vi "get supported types.vi"(8 "error in":errorcluster, 11 "module configuration in":refnum<class "base TBM sequencer configuration.lvclass">) -> (0 "error out":errorcluster, 2 "supported types":T1[](array[typedef]), 3 "module configuration out":refnum<class "base TBM sequencer configuration.lvclass">)   [LabVIEW 2015, in "base TBM sequencer configuration.lvclass"]
doc: "Provides an interface for determining the targets supported by a given configuration/runtime class pairing. This should be overridden by any useful child class."
uses:
  base TBM sequencer configuration.lvclass
  <vilib>/NI/Tag Bus/tag/Data Type.ctl
  <vilib>/NI/Tag Bus Module Framework/module configuration/TBM module configuration.lvclass
  <vilib>/NI/Tag Bus/tag/tag descriptor.lvclass
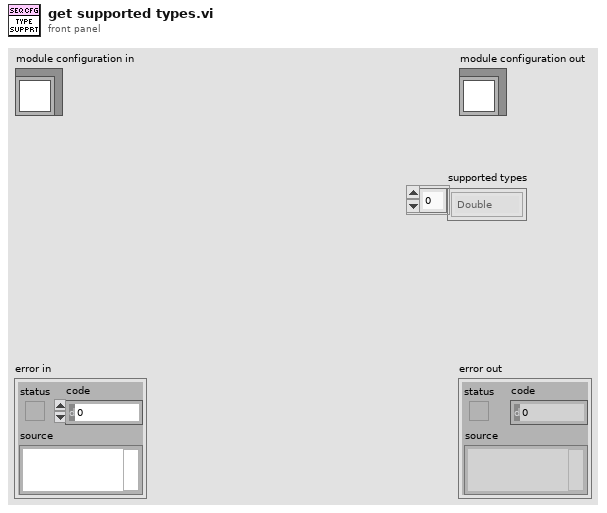
[diagram p1: front panel]
types:
  T1 = typedef "tag bus.lvlib/tag descriptor.lvclass/Data Type.ctl" = enum16{"Double", "Single", "I64", "I32", "I16", "I8", "U64", "U32", "U16", "U8", "Boolean", "String", "Array of Double", "Array of Single", "Array of I64", "Array of I32", "Array of I16", "Array of I8", "Array of U64", "Array of U32", "Array of U16", "Array of U8", "Array of Boolean", "Array of String"}
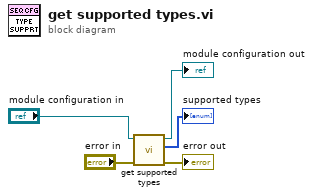
[diagram p0: block diagram]
diagram:
  n1 = call-parent "get supported types.vi"("error in"="error in", "module configuration in"="module configuration in") -> ("error out"=→"error out":errorcluster, "supported types"=→"supported types":T1[], "module configuration out"=→"module configuration out":refnum<class "base TBM sequencer configuration.lvclass">)  [unwired: 7 in]
